vi "Load Picture.vi"(8 "error in (no error)":errorcluster, 11 "Picture Config":T1) -> (0 "error out":errorcluster, 3 "Picture from File":picture)   [LabVIEW 2017]
uses:
  Picture Configuration.ctl
  <vilib>/picture/picture.llb/imagedata.ctl
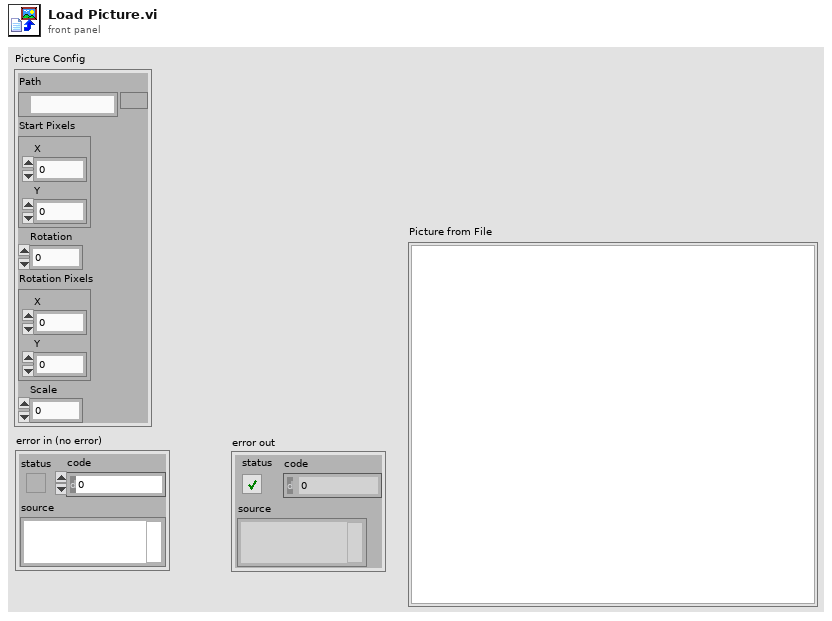
[diagram p1: front panel]
types:
  T1 = typedef "Picture Configuration.ctl" = cluster{"Path":path, "Start Pixels":cluster{"X":i32, "Y":i32}, "Rotation":dbl, "Rotation Pixels":cluster{"X":i32, "Y":i32}, "Scale":dbl}
  T2 = cluster{"left":i16, "top":i16, "right":i16, "bottom":i16}
  T3 = typedef "imagedata.ctl" = cluster{"image type":i32, "image depth":i32, "image":u8[], "mask":u8[], "colors":u32[], "Rectangle":cluster{"left":i16, "top":i16, "right":i16, "bottom":i16}}
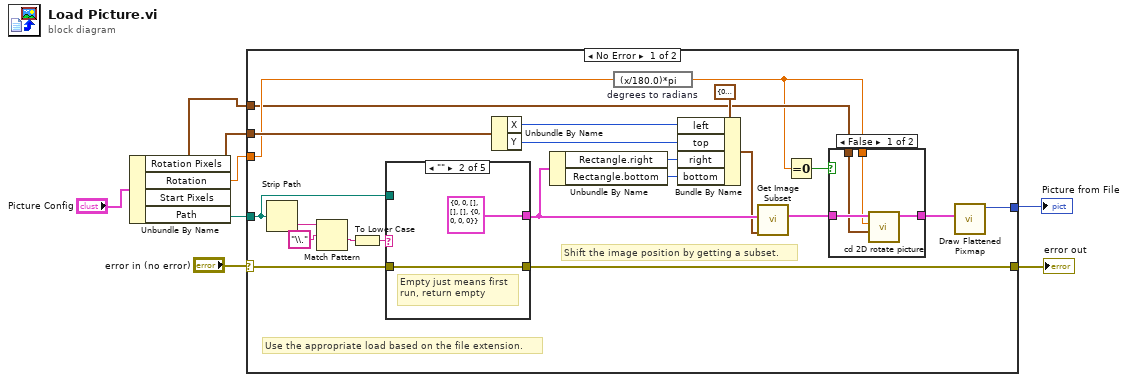
[diagram p0: block diagram]
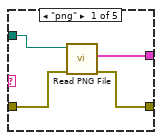
[diagram p3: hidden frame]
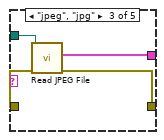
[diagram p4: hidden frame]
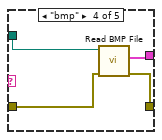
[diagram p5: hidden frame]
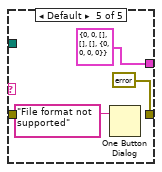
[diagram p6: hidden frame]
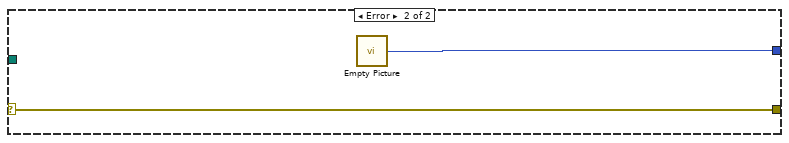
[diagram p7: hidden frame]
diagram:
  n1 = Unbundle By Name("Picture Config") -> ("Rotation Pixels"=w1:cluster{"X":i32, "Y":i32}, "Rotation"=w2:dbl, "Start Pixels"=w3:cluster{"X":i32, "Y":i32}, "Path"=w4:path)
  n2 = case shown="No Error" "error in (no error)" {
    selector: "error in (no error)" -> [w25 w54]
    tunnel: w4 -> [w24 _]
    tunnel: [w27 w53] -> w8
    tunnel: [w26 w54] -> w7
    tunnel: w3 -> [w22 _]
    tunnel: w2 -> [w14 _]
    tunnel: w1 -> [w11 _]
    frame No Error {
      # "Shift the image position by getting a subset."
      # "Use the appropriate load based on the file extension."
      n3 = Strip Path(path=w24) -> (name=w30:string)  [unwired: 1 out]
      n4 = Match Pattern(string=w30, regular expression="\\.") -> (after substring=w28:string)  [unwired: 1 in, 3 out]
      n5 = To Lower Case(string=w28) -> (all lower case string=w23:string)
      n6 = case shown="\"\"" w23 {
        tunnel: w24 -> [w39 _ w45 w47 _]
        tunnel: [w38 w40 w43 w49 errorcluster {"status"=FALSE, "code"=0, "source"=""} ("error out")] -> w26
        tunnel: [w37 T3 {"image type"=0, "image depth"=0, "image"=[], "mask"=[], "colors"=[], "Rectangle"={"left"=0, "top"=0, "right"=0, "bottom"=0}} ("image data") w44 w48 T3 {"image type"=0, "image depth"=0, "image"=[], "mask"=[], "colors"=[], "Rectangle"={"left"=0, "top"=0, "right"=0, "bottom"=0}} ("image data")] -> w21
        tunnel: w25 -> [w36 w40 w42 w46 _]
        frame "png" {
          n7 = call <vilib>:"Read PNG File.vi"("error in (no error)"=w36, "path to PNG file"=w39) -> ("error out"=w38:errorcluster, "image data"=w37:T3)  [unwired: 7 in, 1 out]
        }
        frame "" {
          # "Empty just means first\nrun, return empty"
        }
        frame "jpeg", "jpg" {
          n8 = call <vilib>:"Read JPEG File.vi"("error in (no error)"=w42, "path to JPEG file"=w45) -> ("error out"=w43:errorcluster, "image data"=w44:T3)  [unwired: 7 in, 1 out]
        }
        frame "bmp" {
          n9 = call <vilib>:"Read BMP File.vi"("error in (no error)"=w46, "path to BMP file"=w47) -> ("error out"=w49:errorcluster, "image data"=w48:T3)  [unwired: 7 in, 1 out]
        }
        frame Default {
          n10 = One Button Dialog(message="File format not supported") -> ()  [unwired: 1 in, 1 out]
        }
      }
      n11 = Unbundle By Name(w22) -> ("X"=w19:i32, "Y"=w18:i32)
      n12 = Unbundle By Name(w21) -> ("Rectangle.right"=w17:i16, "Rectangle.bottom"=w16:i16)
      n13 = expression code="(x/180.0)*pi" "degrees to radians"(w14) -> (w10:dbl)
      n14 = Bundle By Name(cluster=T2 {"left"=0, "top"=0, "right"=0, "bottom"=0} ("subset rect"), "left"=w19, "top"=w18, "right"=w17, "bottom"=w16) -> (w15:T2)
      n15 = call <vilib>:"Get Image Subset.vi"("subset rect"=w15, "image data"=w21) -> ("image subset"=w13:T3)  [unwired: 4 in, 1 out]
      n16 = Equal To 0?(x=w10) -> (x = 0?=w9:bool)
      n17 = case shown="False" w9 {
        tunnel: w13 -> [w34 w35]
        tunnel: [w33 w35] -> w12
        tunnel: w11 -> [w32 _]
        tunnel: w10 -> [w31 _]
        frame False {
          n18 = call <vilib>:"cd 2D rotate picture.vi"("Center of rotation"=w32, "Angle (deg)"=w31, "image in"=w34) -> ("image out"=w33:T3)  [unwired: 8 in]
        }
        frame True {
        }
      }
      n19 = call <vilib>:"Draw Flattened Pixmap.vi"("image data"=w12) -> ("new picture"=w27:picture)  [unwired: 8 in]
    }
    frame Error {
      n20 = call "Empty Picture"() -> ("empty picture"=w53:picture)
    }
  }
  "Picture from File" <- w8
  "error out" <- w7
